vi "Process Data.vi"(8 "error in (no error)":errorcluster, 9 "XY Plot":refnum<vi>, 10 "Waveforms":waveform(dbl)[](array[waveform]), 11 "F18 Blowdown":refnum<class "F18 Blowdown.lvclass">) -> (0 "error out":errorcluster, 3 "F18 Blowdown out":refnum<class "F18 Blowdown.lvclass">)   [LabVIEW 2025, in "F18 Blowdown.lvlib" / "F18 Blowdown.lvclass"]
uses:
  F18 Blowdown.lvclass
  Users/Public/Documents/Sandia National Labs/TSS Plugin/Tests/XY Plotter.lvlibp/XY Plotter configuration/XY Plotter configuration.lvclass
  Users/Public/Documents/Sandia National Labs/TSS Plugin/Tests/XY Plotter.lvlibp/XY Plotter configuration/Read XY Plotter.vi
  Users/Public/Documents/Sandia National Labs/TSS Plugin/CEF.lvlibp/serializable configuration/CEF_serializable configuration.lvclass
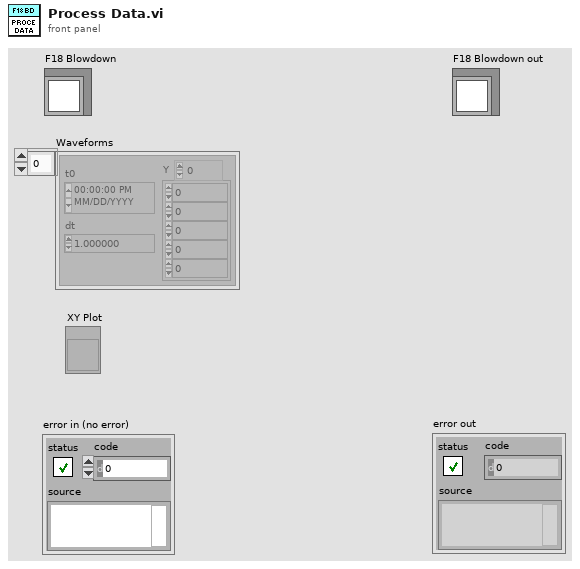
[diagram p1: front panel]
types:
  T1 = typedef "XY Plotter.lvlibp/XY Plotter configuration.lvclass/XY Plotter.ctl" = cluster{"Data Rate":i32, "Y-Scales":cluster{"Label":string, "Max":dbl, "Min":dbl, "Unit":enum16{"---", "V", "mA", "sec", "dB", "deg", "in/s", "in", "lbf", "Hz", "psi", "gpm"}, "Visible":bool}[], "Note":string, "History Length":i32, "DataLog Path":path, "Plot type":bool, "X-Scales":cluster{"Label":string, "Max":dbl, "Min":dbl, "Unit":enum16{"---", "V", "mA", "sec", "dB", "deg", "in/s", "in", "lbf", "Hz", "psi", "gpm"}, "Visible":bool}[], "Plot List":cluster{"Plot Name":string, "X Scale Index":u32, "Y Scale Index":u32, "Visible":bool}[]}
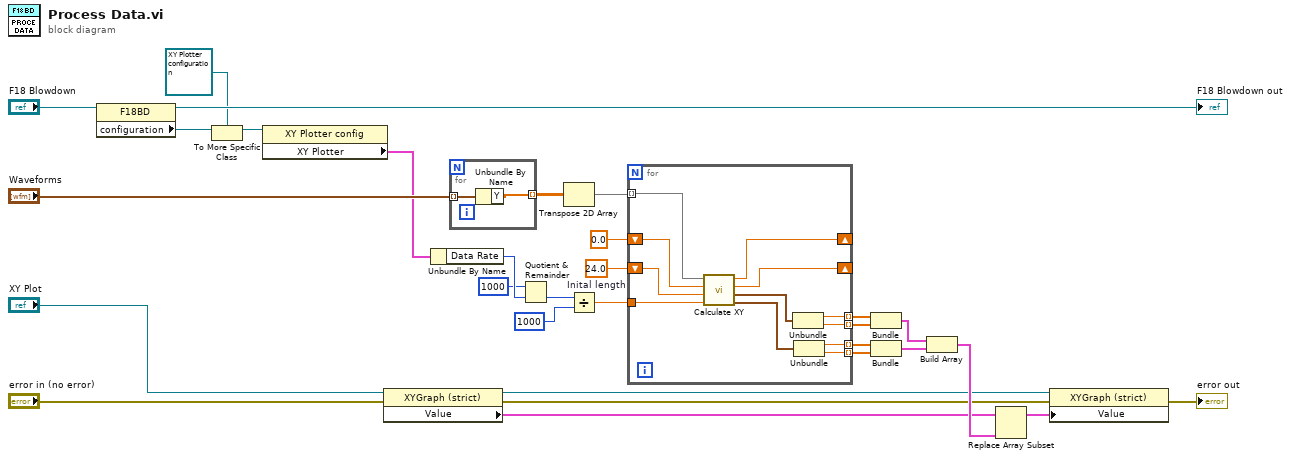
[diagram p0: block diagram]
diagram:
  w15 = 24.0  # Inital length
  n1 = property class="F18BD"(reference="F18 Blowdown") -> (reference out=→"F18 Blowdown out":refnum<class "F18 Blowdown.lvclass">, "configuration"=w7:refnum<class "CEF_serializable configuration.lvclass">)  [unwired: 1 in, 1 out]
  n2 = To More Specific Class(target class=refnum<class "XY Plotter configuration.lvclass"> refnum ("XY Plotter.lvlibp:XY Plotter config"), reference=w7) -> (specific class reference=w8:refnum<class "XY Plotter configuration.lvclass">)  [unwired: 1 in, 1 out]
  n3 = property class="XY Plotter config"(reference=w8) -> ("XY Plotter"=w6:T1)  [unwired: 1 in, 2 out]
  n4 = property class="XYGraph (strict)"(reference="XY Plot", error in="error in (no error)") -> (reference out=w20:refnum<vi>, error out=w19:errorcluster, "Value"=w18:cluster{dbl[], dbl[]}[])
  n5 = Unbundle By Name(w6) -> ("Data Rate"=w5:i32)
  n6 = for {
    tunnel: "Waveforms" -> [w32] mode=indexing
    tunnel: [w31] -> w13 mode=indexing
    n7 = Unbundle By Name(w32) -> ("Y"=w31:dbl[])
  }
  n8 = Quotient & Remainder(x=1000, y=w5) -> (floor(x/y)=w3:i32)  [unwired: 1 out]
  n9 = Transpose 2D Array(2D array=w13) -> (transposed array=w14:dbl[][])
  n10 = Divide(x=w3, y=1000) -> (x/y=w1:dbl)
  n11 = for {
    shift-right: [w44] -> _
    shift-left: 0.0 ("Last High Pressure") -> [w34]
    tunnel: w1 -> [w36]
    shift-right: [w43] -> _
    shift-left: w15 -> [w35]
    tunnel: [w40] -> w24 mode=indexing
    tunnel: [w39] -> w25 mode=indexing
    tunnel: [w38] -> w26 mode=indexing
    tunnel: [w37] -> w27 mode=indexing
    tunnel: w14 -> [w33] mode=indexing
    n12 = call "Calculate XY.vi"("Delta t"=w36, "Last Length"=w35, "Last High Pressure"=w34, "Acquired Data"=w33) -> ("Rate/Force"=w41:cluster{dbl, dbl}, "delP/Flow"=w42:cluster{dbl, dbl}, "Last Length out"=w43:dbl, "Last High Pressure out"=w44:dbl)  [unwired: 4 in]
    n13 = Unbundle(w42) -> (w40:dbl, w39:dbl)
    n14 = Unbundle(w41) -> (w38:dbl, w37:dbl)
  }
  n15 = Bundle(w24, w25) -> (w22:cluster{dbl[], dbl[]})  [unwired: 1 in]
  n16 = Bundle(w26, w27) -> (w23:cluster{dbl[], dbl[]})  [unwired: 1 in]
  n17 = Build Array(w22, w23) -> (w21:cluster{dbl[], dbl[]}[])
  n18 = Replace Array Subset(array=w18, new element=w21) -> (w17:cluster{dbl[], dbl[]}[])  [unwired: 1 in]
  n19 = property class="XYGraph (strict)"(reference=w20, error in=w19, "Value"=w17) -> (error out=→"error out":errorcluster)  [unwired: 1 out]
